vi "FlatToRichfrontend_message.vi"(5 "OutputClusterType":T1, 11 "InputCluster":T2) -> (3 "OutputCluster":T1)   [LabVIEW 2020, in "lexitekDriver_client.lvlib"]
uses:
  lexitekDriver_client.lvlib
  frontend_message_Flat.ctl
  frontend_message.ctl
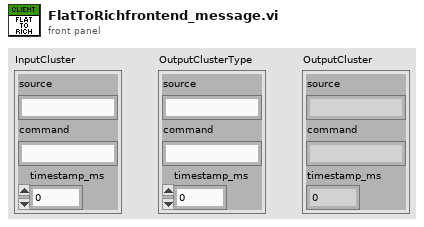
[diagram p1: front panel]
types:
  T1 = typedef "lexitekDriver_client.lvlib/frontend_message.ctl" = cluster{"source":string, "command":string, "timestamp_ms":u64}
  T2 = typedef "lexitekDriver_client.lvlib/frontend_message_Flat.ctl" = cluster{"source":string, "command":string, "timestamp_ms":u64}
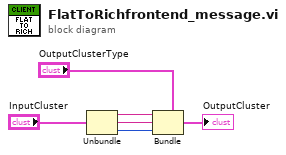
[diagram p0: block diagram]
diagram:
  n1 = Unbundle "Unbundle"("InputCluster") -> ("source"=w3:string, "command"=w2:string, "timestamp_ms"=w1:u64)
  n2 = Bundle "Bundle"(cluster="OutputClusterType", "source"=w3, "command"=w2, "timestamp_ms"=w1) -> (→"OutputCluster":T1)
